vi "PrimaryProviderExample_CreateNewWizard_Interface.vi"() -> (3 "InterfaceTable":T1)   [LabVIEW 2025]
doc: "Tells the Project Explorer provider framework which VIs handle the events of an FRC Subsystem item."
uses:
  <resource>/Framework/Providers/API/CreateNewWizard_Interface.ctl
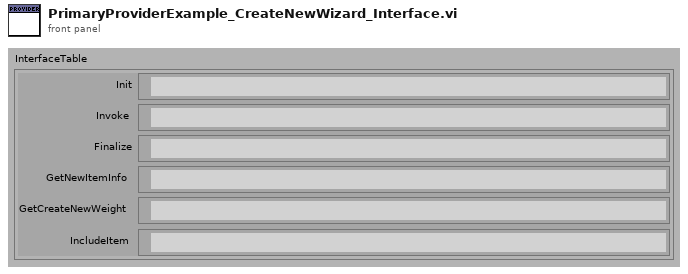
[diagram p1: front panel]
types:
  T1 = typedef "CreateNewWizard_Interface.ctl" = cluster{"Init":path, "Invoke":path, "Finalize":path, "GetNewItemInfo":path, "GetCreateNewWeight":path, "IncludeItem":path}
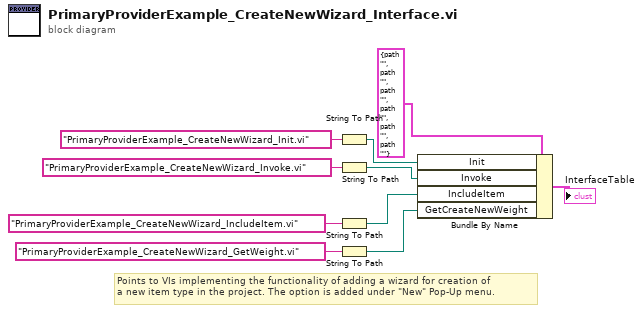
[diagram p0: block diagram]
diagram:
  # "Points to VIs implementing the functionality of adding a wizard for creation of \na new item type in the project. The option is added under \"New\" Pop-Up menu."
  n1 = String To Path(string="PrimaryProviderExample_CreateNewWizard_Init.vi" ("vi path")) -> (path=w8:path)
  n2 = String To Path(string="PrimaryProviderExample_CreateNewWizard_Invoke.vi" ("vi path")) -> (path=w7:path)
  n3 = String To Path(string="PrimaryProviderExample_CreateNewWizard_IncludeItem.vi") -> (path=w4:path)
  n4 = String To Path(string="PrimaryProviderExample_CreateNewWizard_GetWeight.vi") -> (path=w1:path)
  n5 = Bundle By Name(cluster=T1 {"Init"=path "", "Invoke"=path "", "Finalize"=path "", "GetNewItemInfo"=path "", "GetCreateNewWeight"=path "", "IncludeItem"=path ""} ("InterfaceTable"), "Init"=w8, "Invoke"=w7, "IncludeItem"=w4, "GetCreateNewWeight"=w1) -> (→"InterfaceTable":T1)
